vi "get header items from shm clusters.vi"(7 "engine in":refnum<class "Engine Parent Editor Node.lvclass">, 8 "error in (no error)":errorcluster, 10 "shm files":T4[](array[typedef]), 11 "module editor node in":refnum<class "module editor node.lvclass">) -> (0 "error out":errorcluster, 1 "numeric definitions":T1[](array[typedef]), 2 "structs":T3[](array[typedef]), 3 "module editor node out":refnum<class "module editor node.lvclass">, 4 "string definitions":T2[](array[typedef]), 5 "engine out":refnum<class "Engine Parent Editor Node.lvclass">)   [LabVIEW 2014, in "Shared Memory editor node.lvclass"]
uses:
  Shared Memory editor node.lvclass
  <vilib>/NI/DCAF/Tag Editor Core/Configuration Editor/Classes/Module editor node/module editor node.lvclass
  <vilib>/NI/DCAF/Tag Editor Core/Configuration Editor/Classes/Engine Parent/Engine Parent Editor Node.lvclass
  module/configuration/Memory Allocation.ctl
  module/configuration/Line.ctl
  <vilib>/NI/Tag Bus Module Framework/channel/TBM channel.lvclass
  struct params (single type).ctl
  define string params.ctl
  define numeric params.ctl
  module/configuration/Shared Memory configuration.lvclass
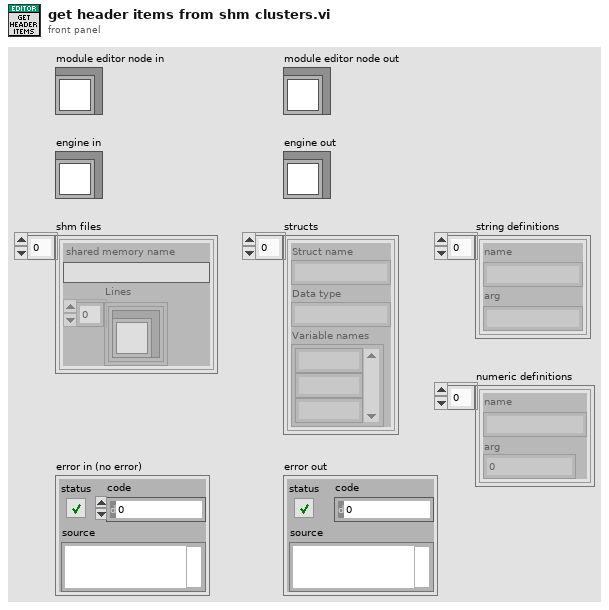
[diagram p1: front panel]
types:
  T1 = typedef "Shared Memory editor node.lvclass/define numeric params.ctl" = cluster{"name":string, "arg":i64}
  T2 = typedef "Shared Memory editor node.lvclass/define string params.ctl" = cluster{"name":string, "arg":string}
  T3 = typedef "Shared Memory editor node.lvclass/struct params (single type).ctl" = cluster{"Struct name":string, "Data type":string, "Variable names":string[]}
  T4 = typedef "Shared Memory configuration.lvclass/Memory Allocation.ctl" = cluster{"shared memory name":string, "Lines":T5[]}
  T5 = typedef "Shared Memory configuration.lvclass/Line.ctl" = cluster{"channel":refnum<class "TBM channel.lvclass">}
  T6 = typedef "tag bus.lvlib/tag descriptor.lvclass/Data Type.ctl" = enum16{"Double", "Single", "I64", "I32", "I16", "I8", "U64", "U32", "U16", "U8", "Boolean", "String", "Array of Double", "Array of Single", "Array of I64", "Array of I32", "Array of I16", "Array of I8", "Array of U64", "Array of U32", "Array of U16", "Array of U8", "Array of Boolean", "Array of String"}
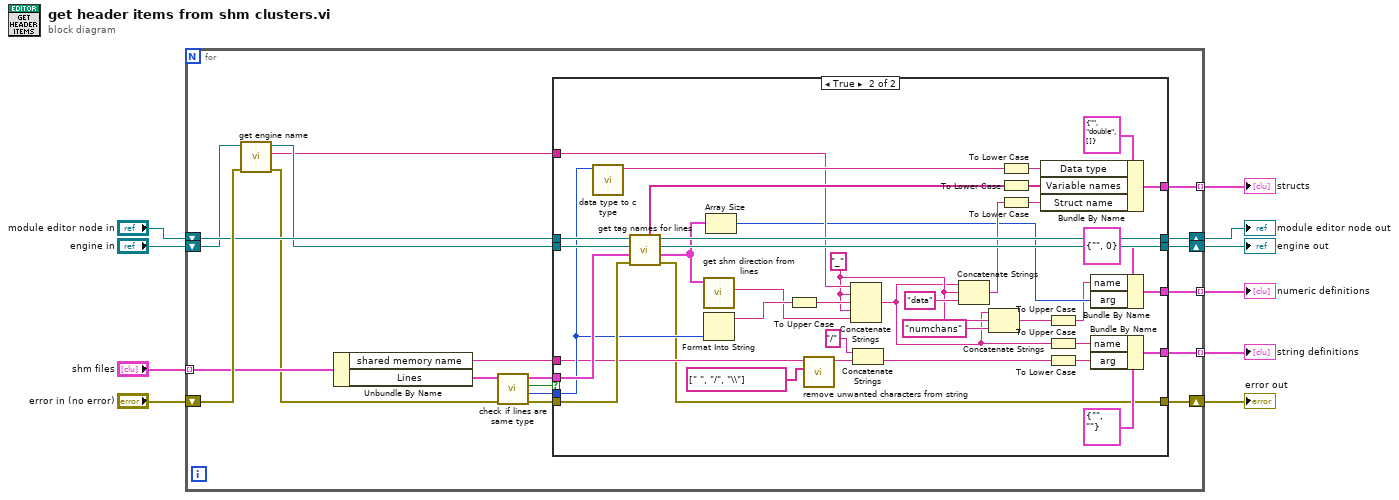
[diagram p0: block diagram]
diagram:
  n1 = for {
    tunnel: "shm files" -> [w28] mode=indexing
    shift-right: [w22] -> w9
    shift-left: "error in (no error)" -> [w29]
    shift-right: [w20] -> w8
    shift-left: "module editor node in" -> [w16]
    shift-right: [w19] -> w7
    shift-left: "engine in" -> [w14]
    tunnel: [w18] -> w3 mode=indexing
    tunnel: [w17] -> w2 mode=indexing
    tunnel: [w11] -> w1 mode=indexing
    n2 = call "get engine name.vi"("error in (no error)"=w29, "engine in"=w14) -> ("error out"=w15:errorcluster, "engine name"=w12:string, "engine out"=w13:refnum<class "Engine Parent Editor Node.lvclass">)  [unwired: 7 in]
    n3 = Unbundle By Name(w28) -> ("shared memory name"=w21:string, "Lines"=w27:T5[])
    n4 = call "check if lines are same type.vi"("error in"=w15, "Lines in"=w27) -> ("error out"=w23:errorcluster, "type"=w24:T6, "all same type?"=w25:bool, "Lines out"=w26:T5[])  [unwired: 6 in]
    n5 = case shown="True" w25 {
      tunnel: w26 -> [_ w70]
      tunnel: w24 -> [_ w61]
      tunnel: w23 -> [w32 w64]
      tunnel: [w32 w36] -> w22
      tunnel: w21 -> [_ w49]
      tunnel: w16 -> [w30 w68]
      tunnel: w13 -> [w31 w67]
      tunnel: [w30 w66] -> w20
      tunnel: [w31 w65] -> w19
      tunnel: [_ w53] -> w18
      tunnel: [_ w52] -> w17
      tunnel: w12 -> [_ w45]
      tunnel: [_ w38] -> w11
      frame False {
        # "Not the same type."
      }
      frame True {
        w40 = "_" ("string")
        n6 = call "data type to c type.vi"("type"=w61) -> ("c type"=w62:string)  [unwired: 10 in]
        n7 = call "get tag names for lines.vi"("error in (no error)"=w64, "Lines in"=w70, "engine in"=w67, "editor node in"=w68) -> ("error out"=w36:errorcluster, "Lines out"=w41:T5[], "engine out"=w65:refnum<class "Engine Parent Editor Node.lvclass">, "editor node out"=w66:refnum<class "module editor node.lvclass">, "tag names"=w69:string[])  [unwired: 3 in]
        n8 = call "get shm direction from lines.vi"("Lines in"=w41) -> ("direction string"=w57:string)  [unwired: 7 in, 3 out]
        n9 = Format Into String(w61) -> (resulting string=w60:string)  [unwired: 3 in, 1 out]
        n10 = Array Size(array=w41) -> (size(s)=w35:i32)
        n11 = To Upper Case(1:w60) -> (0:w59:string)
        n12 = call "remove unwanted characters from string.vi"("unwanted patterns/characters"=string[] [" ", "/", "\\"], "string in"=w49) -> ("string out"=w48:string)  [unwired: 9 in]
        n13 = Concatenate Strings(w45, w40, w59, w40, w57) -> (w37:string)
        n14 = Concatenate Strings("/" ("string"), w48) -> (w46:string)
        n15 = Concatenate Strings(w37, w40, "data" ("string")) -> (w54:string)
        n16 = Concatenate Strings(w37, w40, "numchans" ("string")) -> (w34:string)
        n17 = To Lower Case(string=w62) -> (all lower case string=w63:string)
        n18 = To Lower Case(string=w69) -> (all lower case string=w51:string[])
        n19 = To Lower Case(string=w54) -> (all lower case string=w58:string)
        n20 = Bundle By Name(cluster=T3 {"Struct name"="", "Data type"="double", "Variable names"=[]} ("struct params"), "Data type"=w63, "Variable names"=w51, "Struct name"=w58) -> (w53:T3)
        n21 = To Upper Case(1:w34) -> (0:w33:string)
        n22 = To Upper Case(1:w37) -> (0:w55:string)
        n23 = To Lower Case(string=w46) -> (all lower case string=w50:string)
        n24 = Bundle By Name(cluster=T1 {"name"="", "arg"=0} ("define params"), "name"=w33, "arg"=w35) -> (w38:T1)
        n25 = Bundle By Name(cluster=T2 {"name"="", "arg"=""} ("define params"), "name"=w55, "arg"=w50) -> (w52:T2)
      }
    }
  }
  "module editor node out" <- w8
  "engine out" <- w7
  "error out" <- w9
  "structs" <- w3
  "string definitions" <- w2
  "numeric definitions" <- w1
